vi "Run.vi"(4 "Build Specification Version":T1, 6 "Set PPL Version":bool, 7 "Clear Compiled Object Cache":bool, 8 "error in":errorcluster, 9 "Python Module":path, 10 "Output Folder":path, 11 "IRunner in":refnum<class "IRunner.lvclass">) -> (0 "error out":errorcluster, 3 "IRunner out":refnum<class "IRunner.lvclass">)   [LabVIEW 2026, in "IRunner.lvlib" / "IRunner.lvclass"]
doc: "Run entire generation process through the Runner."
uses:
  IRunner.lvclass
  <vilib>/AppBuilder/AB_API_Simple/Build Specification Version.ctl
  <vilib>/AppBuilder/AB_API_Simple/NI_App_Builder_API.lvlib
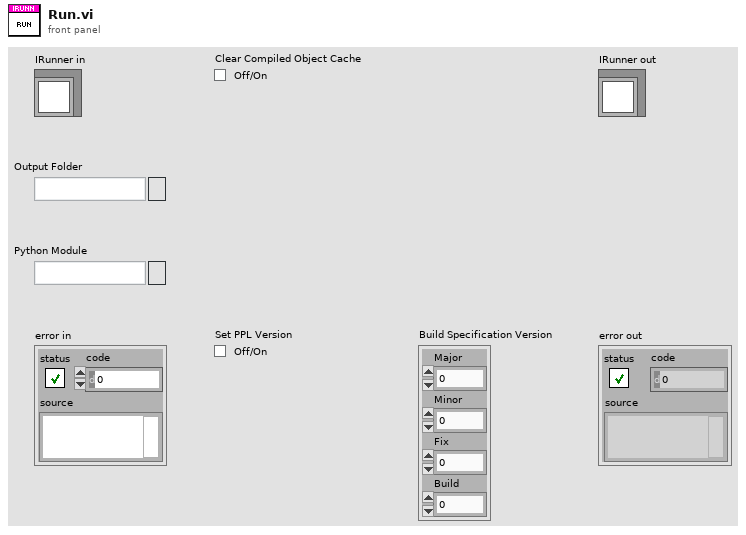
[diagram p1: front panel]
types:
  T1 = typedef "NI_App_Builder_API.lvlib/Build Specification Version.ctl" = cluster{"Major":u16, "Minor":u16, "Fix":u16, "Build":u16}
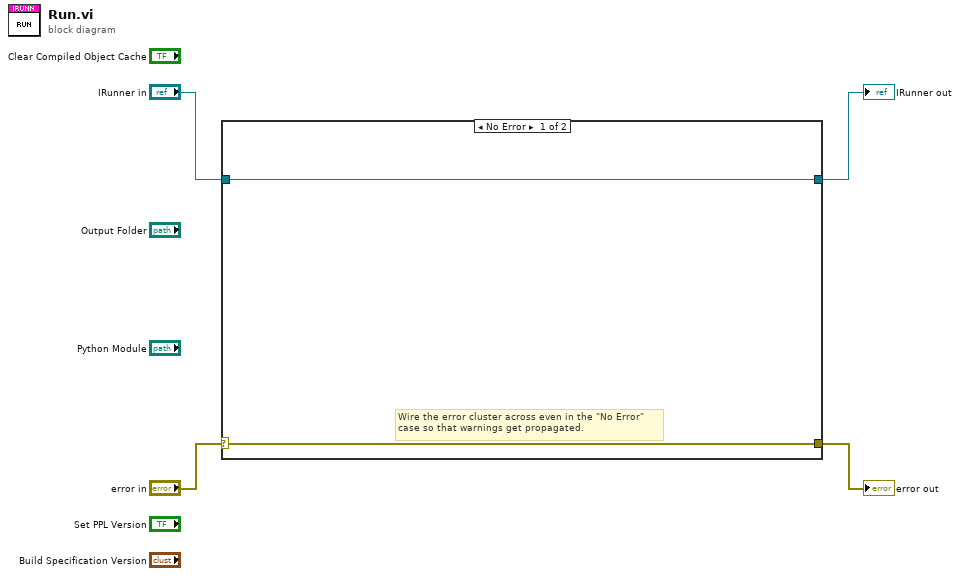
[diagram p0: block diagram]
diagram:
  n1 = case shown="No Error" "error in" {
    selector: "error in" -> [w6 w8]
    tunnel: [w6 w8] -> w3
    tunnel: [w5 w7] -> w1
    tunnel: "IRunner in" -> [w5 w7]
    frame No Error {
      # "Wire the error cluster across even in the \"No Error\"\ncase so that warnings get propagated."
    }
    frame Error {
    }
  }
  "error out" <- w3
  "IRunner out" <- w1
